vi "Set Frequency.vi"(8 "error in (no error)":errorcluster, 10 "Frequency (1000Hz)":dbl=1000.0, 11 "PWM in":refnum<class "LINX-PCA9685 PWM.lvclass">) -> (0 "error out":errorcluster, 3 "PWM out":refnum<class "LINX-PCA9685 PWM.lvclass">)   [LabVIEW 2020, in "LINX-PCA9685 PWM.lvclass"]
doc: "Sets the PWM frequency of the device in Hz."
uses:
  LINX-PCA9685 PWM.lvclass
  LINX I2C/LINX I2C.lvclass
panel:
  out "Prescale Value":dbl
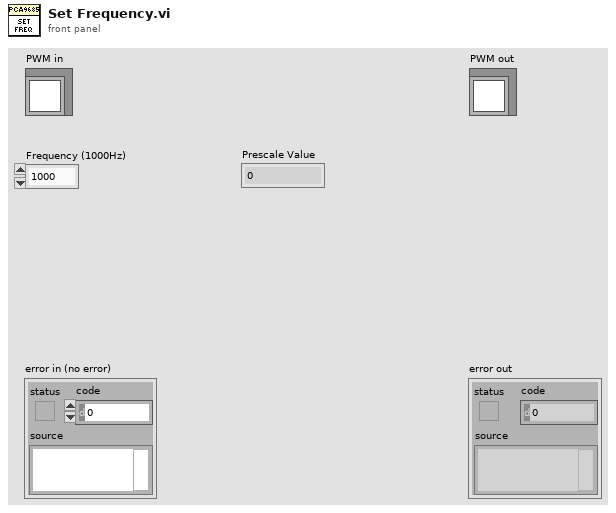
[diagram p1: front panel]
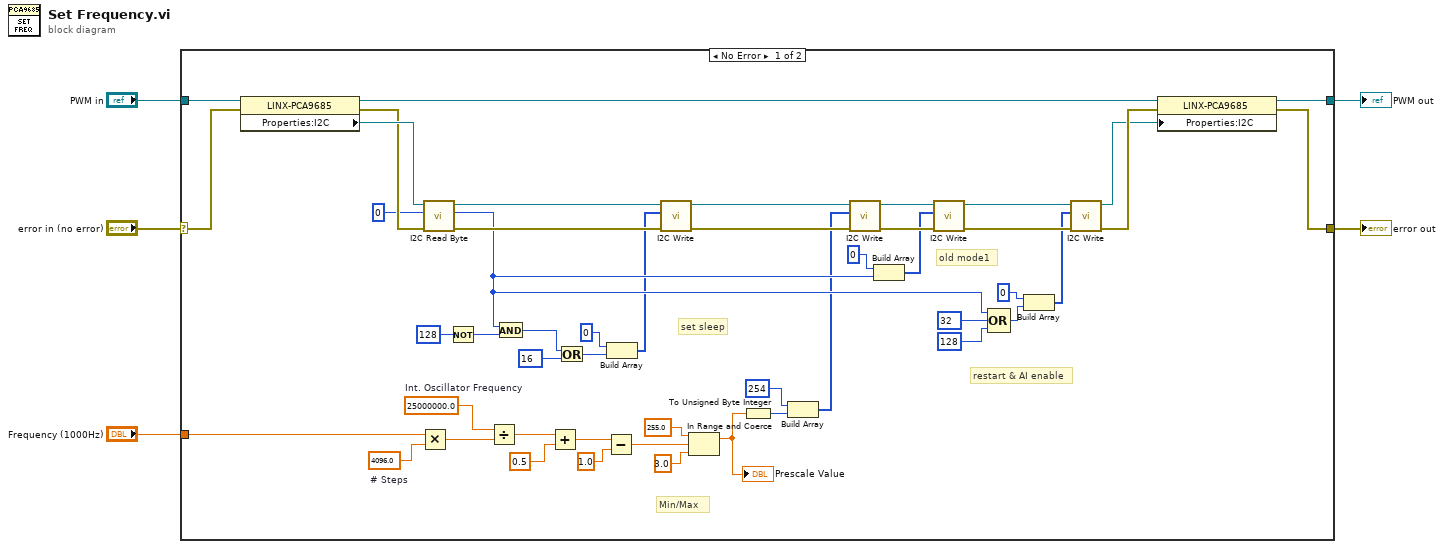
[diagram p0: block diagram]
diagram:
  n1 = case shown="No Error" "error in (no error)" {
    selector: "error in (no error)" -> [w18 w55]
    tunnel: [w12 w55] -> w4
    tunnel: [w11 w54] -> w2
    tunnel: "PWM in" -> [w19 w54]
    tunnel: "Frequency (1000Hz)" -> [w53 _]
    frame No Error {
      w52 = 4096.0  # # Steps
      w51 = 25000000.0  # Int. Oscillator Frequency
      # "set sleep"
      # "old mode1"
      # "restart & AI enable"
      # "Min/Max"
      n2 = property class="LINX-PCA9685"(reference=w19, error in=w18) -> (reference out=w16:refnum<class "LINX-PCA9685 PWM.lvclass">, error out=w15:errorcluster, "Properties:I2C"=w17:refnum<class "LINX I2C.lvclass">)
      n3 = Multiply(x=w53, y=w52) -> (x*y=w50:dbl)
      n4 = call-dynamic "I2C Read Byte.vi"("error in (no error)"=w15, "Register Address"=u8 0 ("Address"), "LINX I2C in"=w17) -> ("error out"=w35:errorcluster, "Byte Read"=w24:u8, "LINX I2C out"=w32:refnum<class "LINX I2C.lvclass">)  [unwired: 6 in]
      n5 = Not(x=u8 128) -> (.not. x?=w38:u8)
      n6 = Divide(x=w51, y=w50) -> (x/y=w49:dbl)
      n7 = And(x=w24, y=w38) -> (x .and. y?=w37:u8)
      n8 = Add(x=w49, y=0.5 ("x")) -> (x+y=w47:dbl)
      n9 = Or(x=w37, y=u8 16) -> (x .or. y?=w30:u8)
      n10 = Subtract(x=w47, y=1.0) -> (x-y=w45:dbl)
      n11 = Build Array(u8 0 ("Address"), w30) -> (w9:u8[])
      n12 = call "I2C Write.vi"("error in (no error)"=w35, "Bytes to Write"=w9, "LINX I2C in"=w32) -> ("error out"=w34:errorcluster, "LINX I2C out"=w33:refnum<class "LINX I2C.lvclass">)  [unwired: 7 in]
      n13 = In Range and Coerce(upper limit=255.0, x=w45, lower limit=3.0) -> (coerced(x)=w42:dbl)  [unwired: 1 out]
      "Prescale Value" <- w42
      n14 = To Unsigned Byte Integer(number=w42) -> (unsigned 8bit integer=w41:u8)
      n15 = Build Array(u8 254 ("unsigned 8bit integer"), w41) -> (w8:u8[])
      n16 = call "I2C Write.vi"("error in (no error)"=w34, "Bytes to Write"=w8, "LINX I2C in"=w33) -> ("error out"=w29:errorcluster, "LINX I2C out"=w28:refnum<class "LINX I2C.lvclass">)  [unwired: 7 in]
      n17 = Build Array(u8 0 ("Address"), w24) -> (w7:u8[])
      n18 = call "I2C Write.vi"("error in (no error)"=w29, "Bytes to Write"=w7, "LINX I2C in"=w28) -> ("error out"=w25:errorcluster, "LINX I2C out"=w26:refnum<class "LINX I2C.lvclass">)  [unwired: 7 in]
      n19 = Compound Arithmetic op=OR(w24, u8 32, u8 128) -> (w20:u8)
      n20 = Build Array(u8 0 ("Address"), w20) -> (w6:u8[])
      n21 = call "I2C Write.vi"("error in (no error)"=w25, "Bytes to Write"=w6, "LINX I2C in"=w26) -> ("error out"=w14:errorcluster, "LINX I2C out"=w13:refnum<class "LINX I2C.lvclass">)  [unwired: 7 in]
      n22 = property class="LINX-PCA9685"(reference=w16, error in=w14, "Properties:I2C"=w13) -> (reference out=w11:refnum<class "LINX-PCA9685 PWM.lvclass">, error out=w12:errorcluster)
    }
    frame Error {
    }
  }
  "error out" <- w4
  "PWM out" <- w2
